vi "guardar_datos.vi"(1 "Path":path=path "C:/Users/cristian/Desktop", 2 "remaining elements":T1[](array[typedef])) -> ()   [LabVIEW 2013]
uses:
  data.ctl
panel:
  out "concatenated string":string
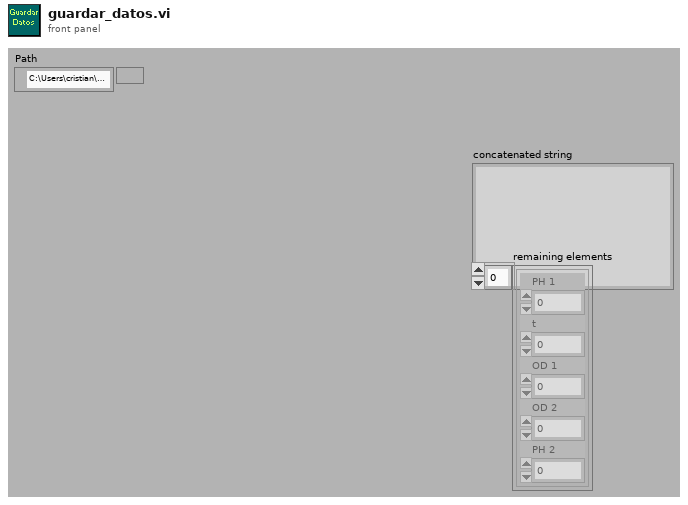
[diagram p1: front panel]
types:
  T1 = typedef "data.ctl" = cluster{"PH 1":dbl, "t":dbl, "OD 1":dbl, "OD 2":dbl, "PH 2":dbl}
  T2 = enum16{"open", "replace", "create", "open or create", "replace or create", "replace or create with confirmation"}
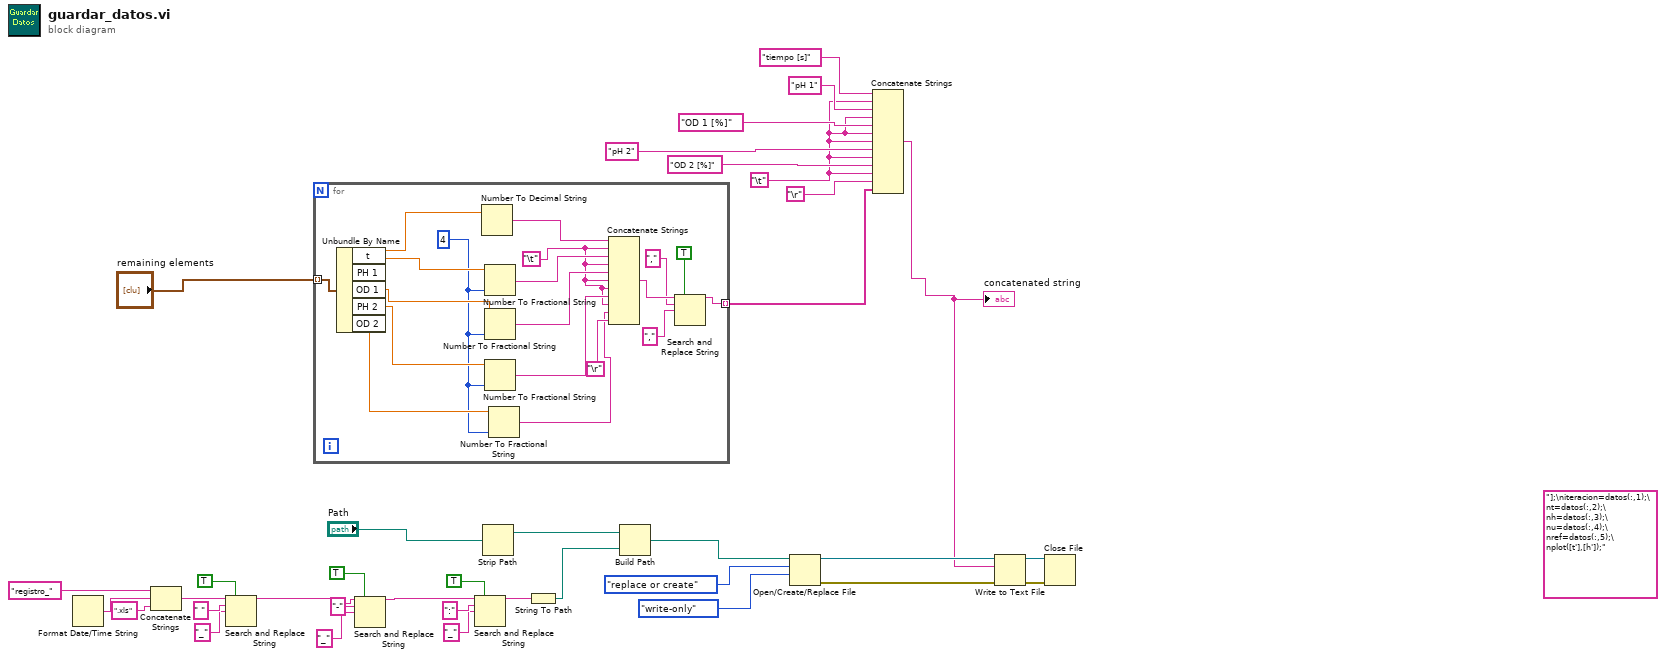
[diagram p0: block diagram]
diagram:
  w1 = "\t"
  (unwired) "];\niteracion=datos(:,1);\nt=datos(:,2);\nh=datos(:,3);\nu=datos(:,4);\nref=datos(:,5);\nplot([t'],[h']);" ("string")
  n1 = Format Date/Time String() -> (date/time string=w27:string)  [unwired: 3 in]
  n2 = Concatenate Strings("registro_" ("string"), w27, ".xls" ("string")) -> (w24:string)
  n3 = Search and Replace String(replace all?=TRUE ("replace all? (F)"), input string=w24, search string=" ", replace string="_" ("replace string (\"\")")) -> (result string=w16:string)  [unwired: 4 in, 3 out]
  n4 = for {
    tunnel: [w50] -> w5 mode=indexing
    tunnel: "remaining elements" -> [w43] mode=indexing
    w38 = "\t"
    w40 = i16 4 ("width (-)")
    n5 = Unbundle By Name(w43) -> ("t"=w46:dbl, "PH 1"=w45:dbl, "OD 1"=w44:dbl, "PH 2"=w42:dbl, "OD 2"=w41:dbl)
    n6 = Number To Decimal String(number=w46) -> (decimal integer string=w55:string)  [unwired: 1 in]
    n7 = Number To Fractional String(number=w45, precision (6)=w40) -> (F-format string=w52:string)  [unwired: 2 in]
    n8 = Number To Fractional String(number=w44, precision (6)=w40) -> (F-format string=w54:string)  [unwired: 2 in]
    n9 = Number To Fractional String(number=w42, precision (6)=w40) -> (F-format string=w39:string)  [unwired: 2 in]
    n10 = Number To Fractional String(number=w41, precision (6)=w40) -> (F-format string=w37:string)  [unwired: 2 in]
    n11 = Concatenate Strings(w55, w38, w52, w38, w54, w38, w38, w39, w38, w37, "\r") -> (w51:string)
    n12 = Search and Replace String(replace all?=TRUE ("replace all? (F)"), input string=w51, search string=",", replace string="," ("replace string (\"\")")) -> (result string=w50:string)  [unwired: 4 in, 3 out]
  }
  n13 = Search and Replace String(replace all?=TRUE ("replace all? (F)"), input string=w16, search string="-", replace string="_" ("replace string (\"\")")) -> (result string=w15:string)  [unwired: 4 in, 3 out]
  n14 = Search and Replace String(replace all?=TRUE ("replace all? (F)"), input string=w15, search string=":", replace string="_" ("replace string (\"\")")) -> (result string=w17:string)  [unwired: 4 in, 3 out]
  n15 = Strip Path(path="Path") -> (stripped path=w30:path)  [unwired: 1 out]
  n16 = String To Path(string=w17) -> (path=w11:path)
  n17 = Build Path(base path=w30, name or relative path=w11) -> (appended path=w29:path)
  n18 = Open/Create/Replace File(file path (use dialog)=w29, operation (0:open)=T2."replace or create", access (0:read/write)=enum16{"read/write", "read-only", "write-only"}."write-only") -> (refnum out=w36:refnum<file>, error out=w34:errorcluster)  [unwired: 3 in, 1 out]
  n19 = Concatenate Strings("tiempo [s]" ("string"), w1, "pH 1" ("string"), w1, "OD 1 [%]" ("string"), w1, w1, "pH 2" ("string"), w1, "OD 2 [%]" ("string"), w1, "\r", w5) -> (w4:string)
  "concatenated string" <- w4
  n20 = Write to Text File(file (use dialog)=w36, text=w4, error in=w34) -> (refnum out=w35:refnum<file>, error out=w33:errorcluster)  [unwired: 1 in, 1 out]
  n21 = Close File(refnum=w35, error in=w33) -> ()  [unwired: 2 out]
